vi "LabApp - Initializing.vi"(6 "error in":errorcluster, 8 "Context Name":string, 9 "variable definitions":T3(array[cluster])=[{"name"="AIData", "alias"="", "type"=enum."1D Array of DBL", "history len"=0}, {"name"="AOData", "alias"="", "type"=enum."1D Array of DBL", "history len"=0}, {"name"="Us", "alias"="Input Voltage", "type"=enum."DBL Number", "history len"=100}, {"name"="Uc", "alias"="Output Voltage", "type"=enum."DBL Number", "history len"=100}, {"name"="I", "alias"="Current", "type"=enum."DBL Number", "history len"=100}, {"name"="Pc", "alias"="Consumed Power", "type"=enum."DBL Number", "history len"=100}]) -> (0 "error out":errorcluster, 3 "VC Handle out":T1)   [LabVIEW 2021]
doc: "::: CalcExpress Toolkit :::\nCopyright (c) 2000-2026 Konstantin Shifershteyn. All rights reserved."
uses:
  vi.lib/addons/CalcExpress/cetypes.llb/CalcExpress Data Type.ctl
  vi.lib/addons/CalcExpress/cetypes.llb/VarMan Variable Context Handle.ctl
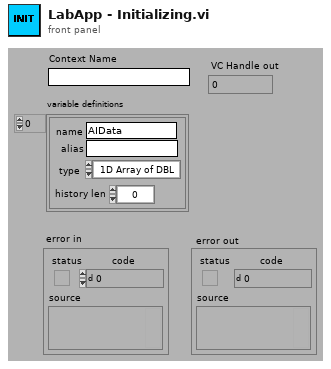
[diagram p1: front panel]
types:
  T1 = typedef "VarMan Variable Context Handle.ctl" = i32
  T2 = typedef "CalcExpress Data Type.ctl" = enum32{"String", "DBL Number", "identifier", "1D Array of DBL", "2D Array of DBL", "CDB Number", "1D Array of CDB", "2D Array of CDB", "1D Array of String", "2D Array of String", "Unknown data type"}
  T3 = cluster{"name":string, "alias":string, "type":T2, "history len":i32}[]
  T4 = enum32{"nothing", "reset", "assign name", "get name", "get handle"}
  T5 = enum16{"create", "destroy", "set value", "get value"}
  T6 = enum32{"nop", "create", "destroy", "reset", "get info", "config"}
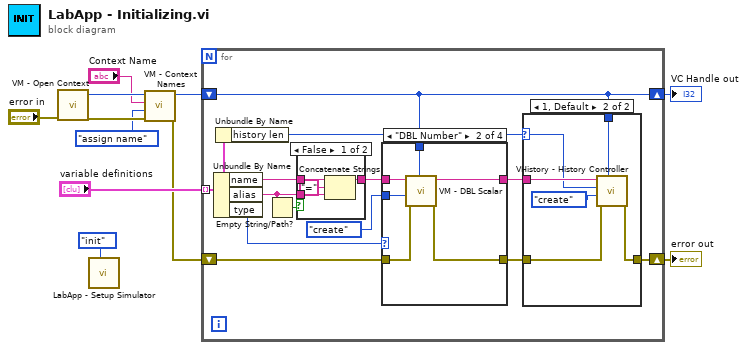
[diagram p0: block diagram]
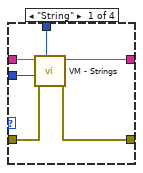
[diagram p3: hidden frame]
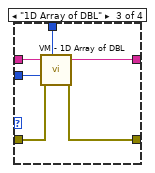
[diagram p4: hidden frame]
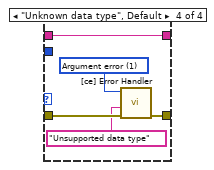
[diagram p5: hidden frame]
diagram:
  n1 = call "VM - Open Context.vi"("error in"="error in") -> ("error out"=w10:errorcluster, "VC Handle out"=w11:T1)  [unwired: 8 in, 1 out]
  n2 = call "LabApp - Setup Simulator.vi"("cmd"=enum16{"init", "get", "set"}."init") -> ()  [unwired: 7 in, 2 out]
  n3 = call "VM - Context Names.vi"("error in"=w10, "action"=T4."assign name", "VC Name"="Context Name", "VC Handle"=w11) -> ("error out"=w5:errorcluster, "VC Handle out"=w7:T1)  [unwired: 2 in, 2 out]
  n4 = for {
    shift-right: [w12] -> w2
    shift-left: w7 -> [w12]
    tunnel: "variable definitions" -> [w21] mode=indexing
    shift-right: [w14] -> w3
    shift-left: w5 -> [w18]
    n5 = Unbundle By Name(w21) -> ("name"=w22:string, "alias"=w23:string, "type"=w17:T2)
    n6 = Unbundle By Name(w21) -> ("history len"=w16:i32)
    n7 = Empty String/Path?(string/path=w23) -> (empty?=w24:bool)
    n8 = case shown="False" w24 {
      tunnel: w23 -> [w57 _]
      tunnel: w22 -> [w58 w59]
      tunnel: [w55 w59] -> w20
      frame False {
        n9 = Concatenate Strings(w58, "=", w57) -> (w55:string)
      }
      frame True {
      }
    }
    n10 = case shown="\"DBL Number\"" w17 {
      tunnel: w20 -> [w37 w42 w49 w54]
      tunnel: T5."create" ("cmd") -> [w33 w41 w48 _]
      tunnel: w18 -> [w36 w40 w47 w52]
      tunnel: [w35 w39 w45 w53] -> w15
      tunnel: w12 -> [w34 w43 w46 _]
      tunnel: [w32 w38 w44 w54] -> w13
      frame "String" {
        n11 = call "VM - Strings.vi"("VC Handle"=w34, "error in"=w36, "cmd"=w33, "name_spec"=w37) -> ("error out"=w35:errorcluster, "dup name_spec"=w32:string)  [unwired: 2 in, 4 out]
      }
      frame "DBL Number" {
        n12 = call "VM - DBL Scalar.vi"("VC Handle"=w43, "error in"=w40, "cmd"=w41, "name_spec"=w42) -> ("error out"=w39:errorcluster, "dup name_spec"=w38:string)  [unwired: 2 in, 4 out]
      }
      frame "1D Array of DBL" {
        n13 = call "VM - 1D Array of DBL.vi"("VC Handle"=w46, "error in"=w47, "cmd"=w48, "name_spec"=w49) -> ("error out"=w45:errorcluster, "dup name_spec"=w44:string)  [unwired: 2 in, 4 out]
      }
      frame "Unknown data type", Default {
        w51 = u16 1 items=["No error", "Argument error", "Memory is full", "Out of zone", "End of file", "File already open", "Generic file I/O error", "File not found", "File permission error", "Disk is full", "Duplicate path", "Too many files open", "System feature not enabled", "Resource file not found", "Cannot add resource", "Resource not found", "Image not found", "Image memory error", "Pen does not exist", "Config type invalid", "Config token not found", "Config parse error", "Config memory error", "Bad external code format", "Bad external code offset", "External code not present", "Null window", "Destroy window error", "Null menu", "Print aborted", "Bad print record", "Print driver error", "Windows error during printing", "Memory error during printing", "Print dialog error", "Generic print error", "Invalid device refnum", "Device not found", "Device parameter error", "Device unit error", "Cannot open device", "Device call aborted", "Generic error", "Cancelled by user", "Object ID too low", "Object ID too high", "Object not in heap", "Unknown heap", "Unknown object (invalid DefProc)", "Unknown object (DefProc not in table)", "Message out of range", "Invalid (null) method", "Unknown message", "Manager call not supported", "Bad address", "Network operation in progress", "Network operation timed out", "Connection is busy", "Network attribute not supported", "Network error", "Address in use", "System out of memory", "Connection aborted", "Connection refused", "Not connected", "Already connected", "Connection closed", "Initialization error (interapplication manager)", "Bad occurrence", "Wait on unbound occurrence handler", "Occurrence queue overflow", "Datalog type conflict", "Unused", "Unrecognized type (interapplication manager)", "Memory corrupt", "Failed to make temporary DLL", "Old CIN version", "Drag socket not found", "Failed to load drop-object", "Failed to register OLE object", "Failed to release OLE object", "Format specifier type mismatch", "Unknown format specifier", "Too few format specifiers", "Too many format specifiers", "Scan failed", "Newer CIN version", "OLE Convert", "Runtime menu error", "Password tampered", "Unknown error code"]
        n14 = call "[ce] Error Handler.vi"("error in"=w52, "error reason"="Unsupported data type", "error code"=w51) -> ("error out"=w53:errorcluster)  [unwired: 7 in, 1 out]
      }
    }
    n15 = case shown="1, Default" w16 {
      selector: w16 -> [_ w30]
      tunnel: w15 -> [w25 w28]
      tunnel: [w25 w27] -> w14
      tunnel: w13 -> [_ w31]
      tunnel: w12 -> [_ w26]
      frame 0 {
      }
      frame 1, Default {
        n16 = call "VHistory - History Controller.vi"("VC Handle"=w26, "error in"=w28, "cmd (nop:default)"=T6."create", "history length"=w30, "name_spec"=w31) -> ("error out"=w27:errorcluster)  [unwired: 3 in, 3 out]
      }
    }
  }
  "error out" <- w3
  "VC Handle out" <- w2
